vi "RFH-save-water_calib.vi"(5 "Save Name":string, 7 "Save Path":path=path "C:/projects/VNA/src/LabVIEW/spike", 8 "error in (no error)":errorcluster, 9 "Water temp":dbl=25.0, 10 "Common Format":T1) -> (0 "error out":errorcluster, 2 "Filepath":path)   [LabVIEW 2020, in "RFH-Reflection_File_Handler.lvlib"]
doc: "Saves a Common Format cluster as a water calibration file with the water temperature, in the given path and name. Returns the file path."
uses:
  RFH-Reflection_File_Handler.lvlib
  RFH-common_data_format.ctl
  <vilib>/Utility/file.llb/Write Delimited Spreadsheet (DBL).vi
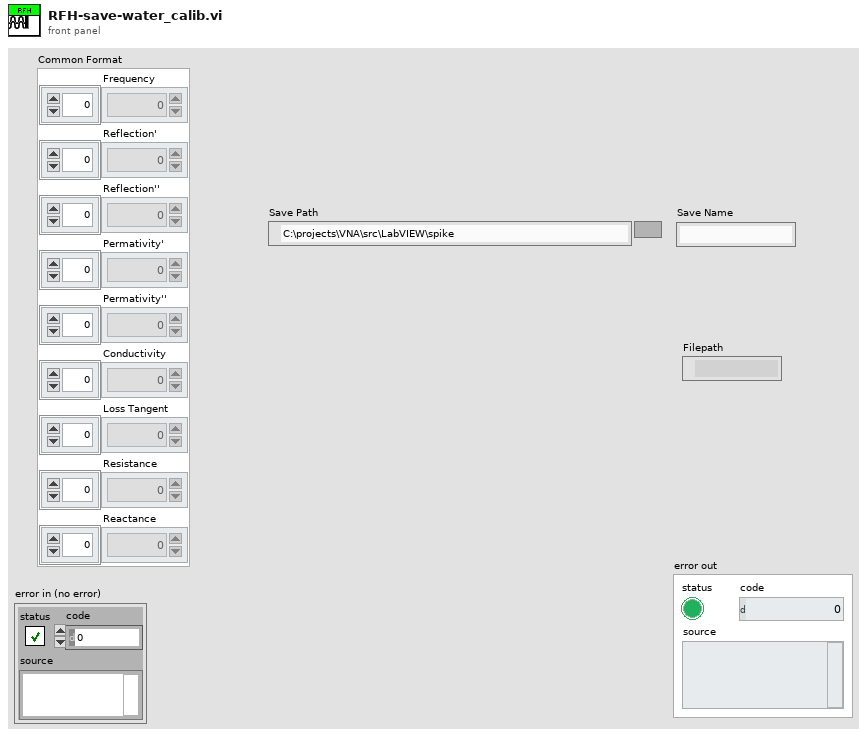
[diagram p1: front panel]
types:
  T1 = typedef "RFH-Reflection_File_Handler.lvlib/RFH-common_data_format.ctl" = cluster{"Frequency":dbl[], "Reflection'":dbl[], "Reflection''":dbl[], "Permativity'":dbl[], "Permativity''":dbl[], "Conductivity":dbl[], "Loss Tangent":dbl[], "Resistance":dbl[], "Reactance":dbl[]}
  T2 = enum16{"open", "replace", "create", "open or create", "replace or create", "replace or create with confirmation"}
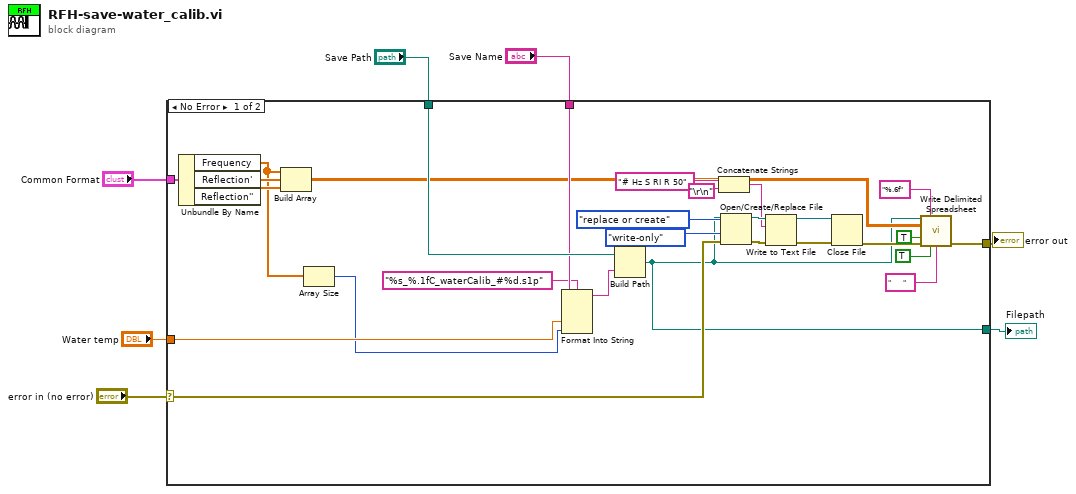
[diagram p0: block diagram]
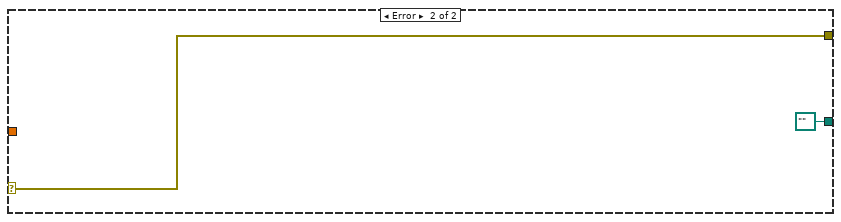
[diagram p2: hidden frame]
diagram:
  n1 = case shown="No Error" "error in (no error)" {
    selector: "error in (no error)" -> [w17 w37]
    tunnel: "Save Path" -> [w35 _]
    tunnel: "Water temp" -> [w21 _]
    tunnel: "Save Name" -> [w20 _]
    tunnel: [w16 w37] -> w3
    tunnel: "Common Format" -> [w12 _]
    tunnel: [w8 path "" ("appended path")] -> w1
    frame No Error {
      n2 = Unbundle By Name(w12) -> ("Frequency"=w11:dbl[], "Reflection'"=w15:dbl[], "Reflection''"=w14:dbl[])
      n3 = Build Array(w11, w15, w14) -> (w13:dbl[][])
      n4 = Array Size(array=w11) -> (size(s)=w10:i32)
      n5 = Format Into String(format string="%s_%.1fC_waterCalib_#%d.s1p", w20, w21, w10) -> (resulting string=w19:string)  [unwired: 2 in, 1 out]
      n6 = Build Path(base path=w35, name or relative path=w19) -> (appended path=w8:path)
      n7 = Concatenate Strings("# Hz S RI R 50" ("text"), "\r\n") -> (w23:string)
      n8 = Open/Create/Replace File(file path (use dialog)=w8, error in=w17, operation (0:open)=T2."replace or create", access (0:read/write)=enum16{"read/write", "read-only", "write-only"}."write-only") -> (refnum out=w28:refnum<file>, error out=w27:errorcluster)  [unwired: 2 in, 1 out]
      n9 = Write to Text File(file (use dialog)=w28, text=w23, error in=w27) -> (refnum out=w30:refnum<file>, error out=w29:errorcluster)  [unwired: 1 in, 1 out]
      n10 = Close File(refnum=w30, error in=w29) -> (error out=w25:errorcluster)  [unwired: 1 out]
      n11 = call-poly <vilib>:"Write Delimited Spreadsheet.vi"("file path (dialog if empty)"=w8, "format (%.3f)"="%.6f", "2D data"=w13, "append to file? (new file:F)"=TRUE, "error in (no error)"=w25, "transpose? (no:F)"=TRUE, "delimiter (\\t)"="      " ("delimiter (\\t)")) -> ("error out"=w16:errorcluster)  [unwired: 7 in, 1 out]
    }
    frame Error {
    }
  }
  "error out" <- w3
  "Filepath" <- w1
